vi "onListenForNewConnection.vi"(8 "error in (no error)":errorcluster, 9 "timeout (ms)":i32=2000, 11 "Listener":refnum<class "Connection.TCP.lvclass">) -> (0 "error out":errorcluster, 1 "New connection":bool, 2 "timed out":bool, 3 "New Connection":refnum<class "Connection.lvclass">)   [LabVIEW 2013, in "Connection.TCP_GOSPL.lvlib" / "Connection.TCP.lvclass"]
uses:
  Connection.TCP.lvclass
  Connection/Connection.lvclass
  Connection.TCP.lvclass/Connection.TCP.ctl
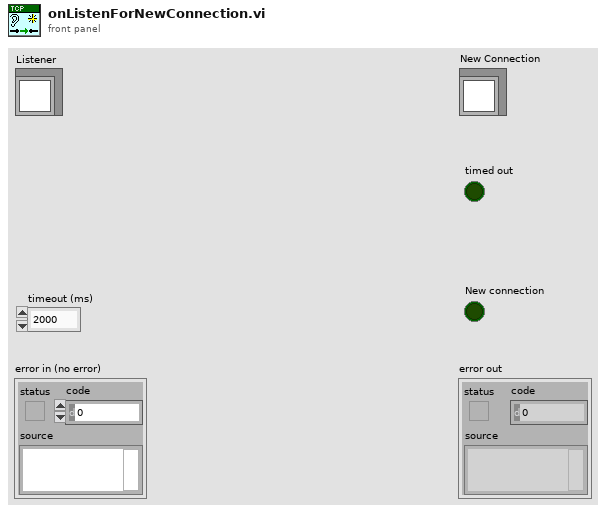
[diagram p1: front panel]
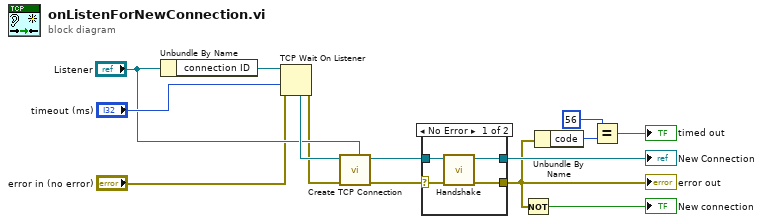
[diagram p0: block diagram]
diagram:
  n1 = Unbundle By Name("Listener") -> ("connection ID"=w13:refnum<k5>)
  n2 = TCP Wait On Listener(8:"error in (no error)", 9:"timeout (ms)", 11:w13) -> (0:w3:errorcluster, 4:w12:refnum<k5>)  [unwired: 1 in, 3 out]
  n3 = call "Create TCP Connection.vi"("Connection.TCP"="Listener", "error in (no error)"=w3, "connection ID"=w12) -> ("error out"=w4:errorcluster, "Connection.TCP"=w1:refnum<class "Connection.TCP.lvclass">)  [unwired: 7 in]
  n4 = case shown="No Error" w4 {
    selector: w4 -> [w15 w20]
    tunnel: w1 -> [w18 w19]
    tunnel: [w17 w19] -> w7
    tunnel: [w16 w20] -> w2
    frame No Error {
      n5 = call-dynamic "Handshake.vi"("error in (no error)"=w15, "Connection in"=w18) -> ("error out"=w16:errorcluster, "Connection out"=w17:refnum<class "Connection.TCP.lvclass">)  [unwired: 8 in]
    }
    frame Error {
    }
  }
  "error out" <- w2
  "New Connection" <- w7
  n6 = Not(x=w2) -> (.not. x?=→"New connection":bool)
  n7 = Unbundle By Name(w2) -> ("code"=w10:i32)
  n8 = Equal?(x=56, y=w10) -> (x = y?=→"timed out":bool)
